vi "Drop_DecodeIncomingPacket.vi"   [LabVIEW 2013]
uses:
  ControlPacket/ControlPacket.lvclass
  MQTT_311/MQTTVersion.lvclass
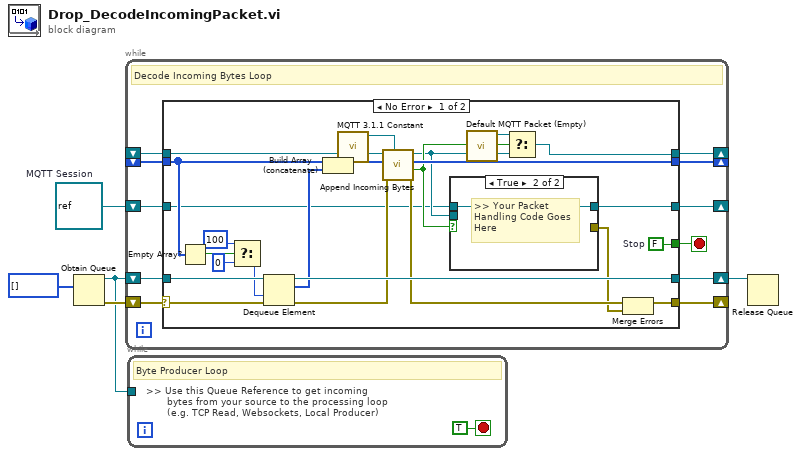
[diagram p0: block diagram]
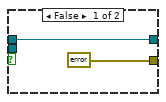
[diagram p2: hidden frame]
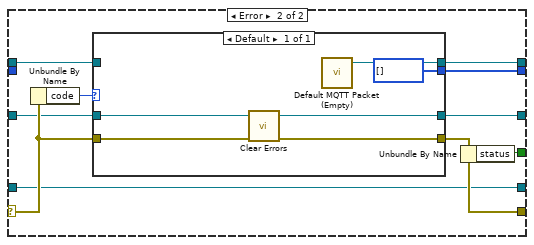
[diagram p3: hidden frame]
diagram:
  w1 = refnum<class> refnum  # MQTT Session
  n1 = Obtain Queue(element data type=u8[] [] ("Remaining Packets")) -> (queue out=w2:refnum<queue>, error out=w5:errorcluster)  [unwired: 4 in, 1 out]
  n2 = while {
    shift-right: [w14] -> _
    shift-left: _ -> [w13]
    shift-right: [w12] -> _
    shift-left: w5 -> [w11]
    shift-right: [w15] -> _
    shift-left: _ -> [w16]
    shift-right: [w8] -> w3
    shift-left: w2 -> [w9]
    shift-right: [w6] -> _
    shift-left: w1 -> [w7]
    stop <- w10 stop-if-true
    # "Decode Incoming Bytes Loop"
    n3 = case shown="No Error" w11 {
      selector: w11 -> [w32 w51]
      tunnel: w16 -> [w40 w49]
      tunnel: [w23 w53] -> w15
      tunnel: [w38 w52] -> w14
      tunnel: w13 -> [w28 _]
      tunnel: [w29 w48] -> w12
      tunnel: [w37 w47] -> w10
      tunnel: w9 -> [w36 w46]
      tunnel: [w35 w46] -> w8
      tunnel: w7 -> [w18 w45]
      tunnel: [w17 w44] -> w6
      frame No Error {
        w37 = FALSE  # Stop
        # "No Error"
        n4 = Empty Array?(array=w28) -> (empty?=w27:bool)
        n5 = Select(t=100 ("timeout in ms (-1)"), s=w27, f=0) -> (s? t:f=w25:i32)
        n6 = Dequeue Element(queue=w36, timeout in ms (-1)=w25, error in (no error)=w32) -> (queue out=w35:refnum<queue>, element=w34:u8[], error out=w31:errorcluster)  [unwired: 1 out]
        n7 = Build Array (concatenate)(w28, w34) -> (w33:u8[])
        n8 = call "MQTT 3.1.1 Constant.vi"() -> ("MQTT 3.1.1"=w39:refnum<class "MQTTVersion.lvclass">)  [unwired: 11 in]
        n9 = call "Append Incoming Bytes.vi"("MQTT Version (3.1.1)"=w39, "error in (no error)"=w31, "Incoming Packets"=w33, "Incomplete ControlPacket"=w40) -> ("error out"=w30:errorcluster, "Complete Packet"=w21:bool, "Remaining Packets"=w38:u8[], "ControlPacket"=w20:refnum<class "ControlPacket.lvclass">)  [unwired: 4 in]
        n10 = case shown="True" w21 {
          tunnel: [errorcluster {"status"=FALSE, "code"=0, "source"=""} ("error out") _] -> w19
          tunnel: w20 -> [_ _]
          tunnel: w18 -> [w41 w43]
          tunnel: [w41 w43] -> w17
          frame False {
            # "No Packet received"
          }
          frame True {
            # ">> Your Packet\nHandling Code Goes Here"
            # "Packet Received"
          }
        }
        n11 = call "Default MQTT Packet (Empty).vi"() -> ("No Packet"=w22:refnum<class "ControlPacket.lvclass">)  [unwired: 11 in]
        n12 = Select(t=w22, s=w21, f=w20) -> (s? t:f=w23:refnum<class "ControlPacket.lvclass">)
        n13 = Merge Errors(w30, w19) -> (w29:errorcluster)
      }
      frame Error {
        # "Handle Error"
        n14 = Unbundle By Name(w51) -> ("code"=w50:i32)
        n15 = case shown="Default" w50 {
          tunnel: [w55] -> w53
          tunnel: w51 -> [w58]
          tunnel: [w57] -> w48
          tunnel: [u8[] [] ("Remaining Packets")] -> w52
          tunnel: w49 -> [_]
          tunnel: w45 -> [w54]
          tunnel: [w54] -> w44
          frame Default {
            # "Malformed Packet"
            n16 = call <vilib>:"Clear Errors.vi"("error in (no error)"=w58) -> ("error out"=w57:errorcluster)  [unwired: 6 in]
            n17 = call "Default MQTT Packet (Empty).vi"() -> ("No Packet"=w55:refnum<class "ControlPacket.lvclass">)  [unwired: 11 in]
          }
        }
        n18 = Unbundle By Name(w48) -> ("status"=w47:bool)
      }
    }
  }
  n19 = while {
    tunnel: w2 -> [_]
    stop <- TRUE stop-if-true
    # ">> Use this Queue Reference to get incoming\n       bytes from your source to the processing loop\n       (e.g. TCP Read, Websockets, Local Producer)"
    # "Byte Producer Loop"
  }
  n20 = Release Queue(queue=w3) -> ()  [unwired: 2 in, 3 out]
